vi "Generate Trace for Disconnected Network Endpoint.vi"   [LabVIEW 2020]
doc: "Generates a DETT User Generated Trace for a network endpoint being connected to other one.\n\n<b>Connection ID</b> can be port, stream name, ..."
uses:
  <resource>/AFDebug/AF Debug.lvlib
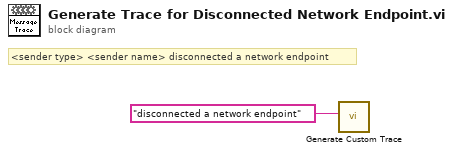
[diagram p0: block diagram]
diagram:
  # "<sender type> <sender name> disconnected a network endpoint"
  n1 = call <resource>:"Generate Custom Trace.vi"("Custom Action"="disconnected a network endpoint" ("input 3")) -> ()  [unwired: 11 in]
